vi "set Reference Level and Atten and Reference Offset.vi"(8 "error in (no error)":errorcluster, 10 "Reference Level, Atten, Reference Offset":T1, 11 "FSV-40N in":refnum<class "FSV-40N.lvclass">) -> (0 "error out":errorcluster, 3 "FSV-40N out":refnum<class "FSV-40N.lvclass">)   [LabVIEW 2023, in "Spectrum Analyzer.lvlib" / "FSV-40N.lvclass"]
uses:
  FSV-40N.lvclass
  TYPE DEFINITION/TYPE Reference Level and Atten Param.ctl
  FSV-40N.lvclass/FSV-40N.ctl
  Spectrum Analyzer.lvlib
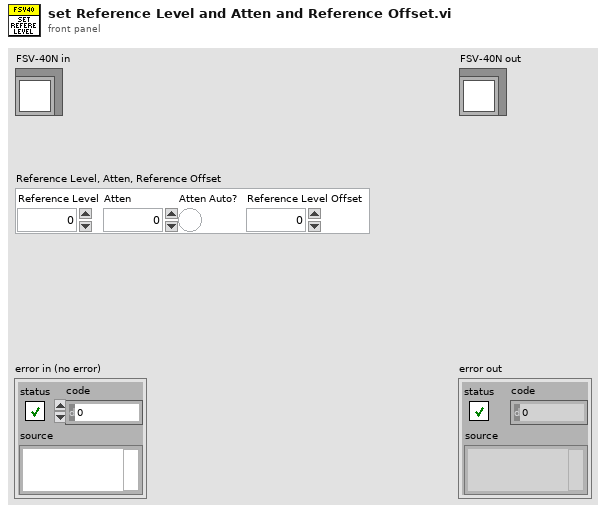
[diagram p1: front panel]
types:
  T1 = typedef "Spectrum Analyzer.lvlib/TYPE Reference Level and Atten Param.ctl" = cluster{"Reference Level":dbl, "Atten":i32, "Atten Auto?":bool, "Reference Level Offset":dbl}
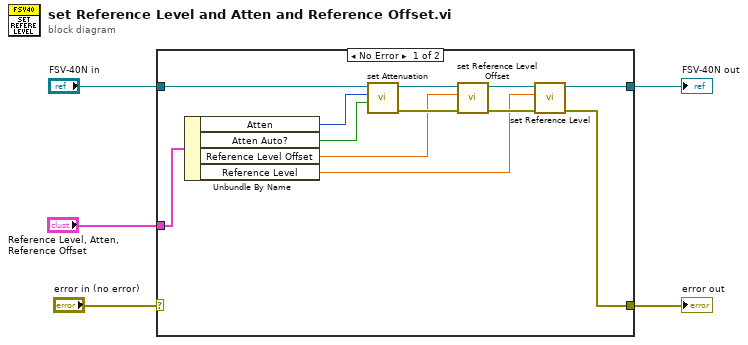
[diagram p0: block diagram]
diagram:
  n1 = case shown="No Error" "error in (no error)" {
    selector: "error in (no error)" -> [_ w18]
    tunnel: "FSV-40N in" -> [w16 w19]
    tunnel: [w7 w19] -> w3
    tunnel: [w6 w18] -> w2
    tunnel: "Reference Level, Atten, Reference Offset" -> [w17 _]
    frame No Error {
      n2 = Unbundle By Name(w17) -> ("Atten"=w13:i32, "Atten Auto?"=w12:bool, "Reference Level Offset"=w11:dbl, "Reference Level"=w8:dbl)
      n3 = call-dynamic "set Attenuation.vi"("Auto?"=w12, "Attenuation"=w13, "FSV-40N in"=w16) -> ("error out"=w14:errorcluster, "FSV-40N out"=w15:refnum<class "FSV-40N.lvclass">)  [unwired: 7 in]
      n4 = call-dynamic "set Reference Level Offset.vi"("error in (no error)"=w14, "Reference Level Offset"=w11, "FSV-40N in"=w15) -> ("error out"=w9:errorcluster, "FSV-40N out"=w10:refnum<class "FSV-40N.lvclass">)  [unwired: 7 in]
      n5 = call-dynamic "set Reference Level.vi"("error in (no error)"=w9, "Reference Level"=w8, "FSV-40N in"=w10) -> ("error out"=w6:errorcluster, "FSV-40N out"=w7:refnum<class "FSV-40N.lvclass">)  [unwired: 7 in]
    }
    frame Error {
    }
  }
  "error out" <- w2
  "FSV-40N out" <- w3
